vi "libssh2_sftp_statvfs.vi"(8 "error in (no error)":errorcluster, 10 "path":string, 11 "sftp":T2) -> (0 "error out":errorcluster, 2 "statvfs":T1)   [LabVIEW 2017, in "libssh2.lvlib"]
doc: "Get the file system information of a file or directory."
uses:
  libssh2.lvlib
  SFTP Refnum.ctl
  libssh2_sftp_statvfs.ctl
  Acquire Session.vi
  Release Session.vi
  Not An SFTP Refnum.vi
  <vilib>/Utility/error.llb/Error Cluster From Error Code.vi
  Global Settings.vi
  Read SFTP Refnum.vi
  Read Session Refnum.vi
  <vilib>/Utility/semaphor.llb/Acquire Semaphore.vi
  <vilib>/Utility/semaphor.llb/Release Semaphore.vi
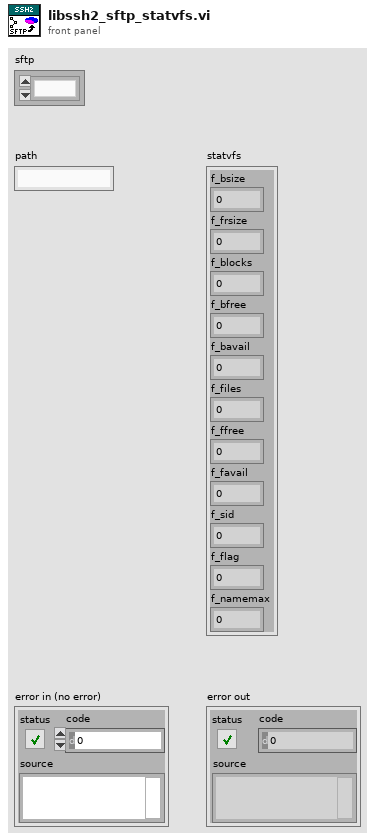
[diagram p1: front panel]
types:
  T1 = typedef "libssh2.lvlib/libssh2_sftp_statvfs.ctl" = cluster{"f_bsize":u64, "f_frsize":u64, "f_blocks":u64, "f_bfree":u64, "f_bavail":u64, "f_files":u64, "f_ffree":u64, "f_favail":u64, "f_sid":u64, "f_flag":u64, "f_namemax":u64}
  T2 = typedef "libssh2.lvlib/SFTP Refnum.ctl" = refnum<k1>
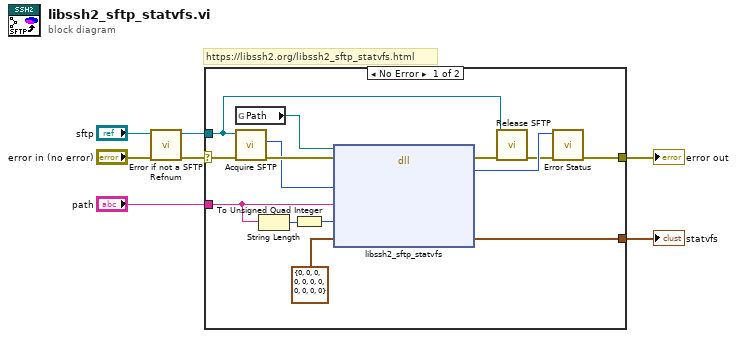
[diagram p0: block diagram]
diagram:
  # "https://libssh2.org/libssh2_sftp_statvfs.html"
  n1 = call "Error if not a SFTP Refnum.vi"("error in (no error)"="error in (no error)", "sftp"="sftp") -> ("error out"=w6:errorcluster, "sftp out"=w5:T2)  [unwired: 8 in]
  n2 = case shown="No Error" w6 {
    selector: w6 -> [w20 w22]
    tunnel: w5 -> [w8 _]
    tunnel: [w16 w22] -> w4
    tunnel: "path" -> [w13 _]
    tunnel: [w11 _] -> w1
    frame No Error {
      n3 = global read "Global Settings.vi" "Path"() -> (w21:path)
      n4 = call "Acquire SFTP.vi"("error in (no error)"=w20, "sftp"=w8) -> ("error out"=w19:errorcluster, "LIBSSH2_SFTP*"=w18:u64)  [unwired: 8 in]
      n5 = String Length(string=w13) -> (length=w14:i32)
      n6 = To Unsigned Quad Integer(1:w14) -> (0:w10:u64)
      n7 = dll-call lib="?" fn="libssh2_sftp_statvfs"(path in=w21, error in=w19, "sftp"=w18, "path"=w13, "path_len"=w10, "st"=T1 {"f_bsize"=0, "f_frsize"=0, "f_blocks"=0, "f_bfree"=0, "f_bavail"=0, "f_files"=0, "f_ffree"=0, "f_favail"=0, "f_sid"=0, "f_flag"=0, "f_namemax"=0} ("statvfs")) -> (error out=w17:errorcluster, "return value"=w15:i32, "st"=w11:T1)  [unwired: 4 in, 1 out]
      n8 = call "Release SFTP.vi"("error in (no error)"=w17, "sftp"=w8) -> ("error out"=w9:errorcluster)  [unwired: 9 in]
      n9 = call "Error Status.vi"("error in (no error)"=w9, "return value"=w15) -> ("error out"=w16:errorcluster)  [unwired: 8 in, 1 out]
    }
    frame Error {
    }
  }
  "error out" <- w4
  "statvfs" <- w1
